vi "VM Spy - probe file name & win title.vi"(8 "Variable":string, 9 "VC Handle":T1=-1) -> (1 "alias":string, 2 "var name":string, 3 "VC Handle out":T1=-1, 4 "probe win title":string, 5 "probe instance name":string)   [LabVIEW 2021]
doc: "::: CalcExpress Toolkit :::\nCopyright (c) 2000-2026 Konstantin Shifershteyn. All rights reserved."
uses:
  vi.lib/addons/CalcExpress/cetypes.llb/VarMan Variable Context Handle.ctl
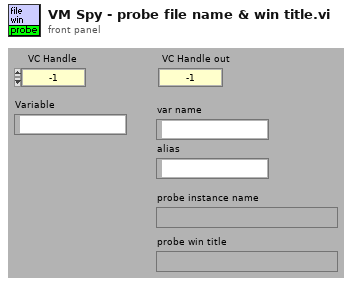
[diagram p1: front panel]
types:
  T1 = typedef "VarMan Variable Context Handle.ctl" = i32
  T2 = enum32{"nothing", "reset", "assign name", "get name", "get handle"}
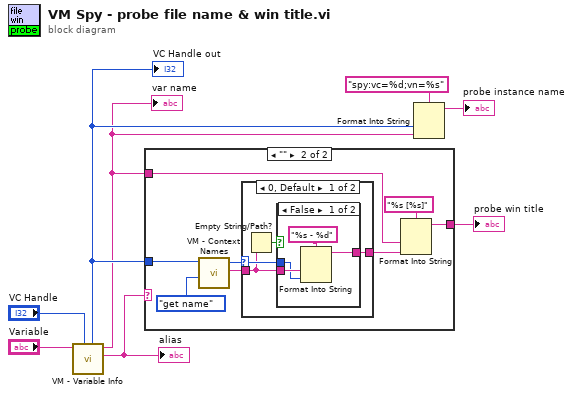
[diagram p0: block diagram]
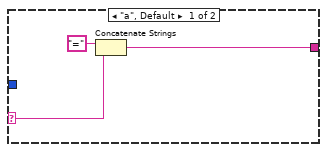
[diagram p2: hidden frame]
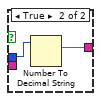
[diagram p3: hidden frame]
diagram:
  n1 = call "VM - Variable Info.vi"("VC Handle"="VC Handle", "name_spec"="Variable") -> ("alias"=w5:string, "var name"=w1:string, "var VC Handle"=w2:T1)  [unwired: 4 in, 3 out]
  "var name" <- w1
  "VC Handle out" <- w2
  "alias" <- w5
  n2 = case shown="\"\"" w5 {
    selector: w5 -> [w10 _]
    tunnel: [w11 w13] -> w6
    tunnel: w2 -> [_ w14]
    tunnel: w1 -> [_ w12]
    frame "a", Default {
      n3 = Concatenate Strings("=", w10) -> (w11:string)
    }
    frame "" {
      n4 = call "VM - Context Names.vi"("action"=T2."get name", "VC Handle"=w14) -> ("VC Name out"=w17:string, "VC Handle out"=w18:T1)  [unwired: 4 in, 2 out]
      n5 = case shown="0, Default" w18 {
        selector: w18 -> [w21 _]
        tunnel: [w22 w30] -> w19
        tunnel: w17 -> [w20 w30]
        frame 0, Default {
          n6 = Empty String/Path?(string/path=w20) -> (empty?=w23:bool)
          n7 = case shown="False" w23 {
            tunnel: w20 -> [w26 _]
            tunnel: w21 -> [w25 w28]
            tunnel: [w24 w29] -> w22
            frame False {
              n8 = Format Into String(format string="%s - %d", w26, w25) -> (resulting string=w24:string)  [unwired: 2 in, 1 out]
            }
            frame True {
              n9 = Number To Decimal String(number=w28) -> (decimal integer string=w29:string)  [unwired: 1 in]
            }
          }
        }
        frame -1 {
        }
      }
      n10 = Format Into String(format string="%s [%s]", w12, w19) -> (resulting string=w13:string)  [unwired: 2 in, 1 out]
    }
  }
  "probe win title" <- w6
  n11 = Format Into String(format string="spy:vc=%d;vn=%s", w2, w1) -> (resulting string=→"probe instance name":string)  [unwired: 2 in, 1 out]
